vi "P5_PrintVIToHTML.vi"(11 "Inputs":string[](array[string])) -> (2 "Output/Failure":string, 3 "CLI Process Return Code":i32)   [LabVIEW 2026]
doc: "Slice 1.1 probe: Open VI Reference, Print VI To HTML to the path in arg, close the reference."
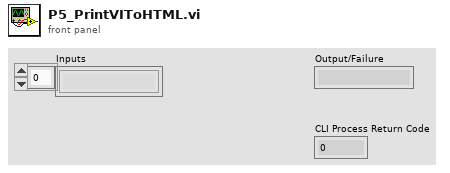
[diagram p1: front panel]
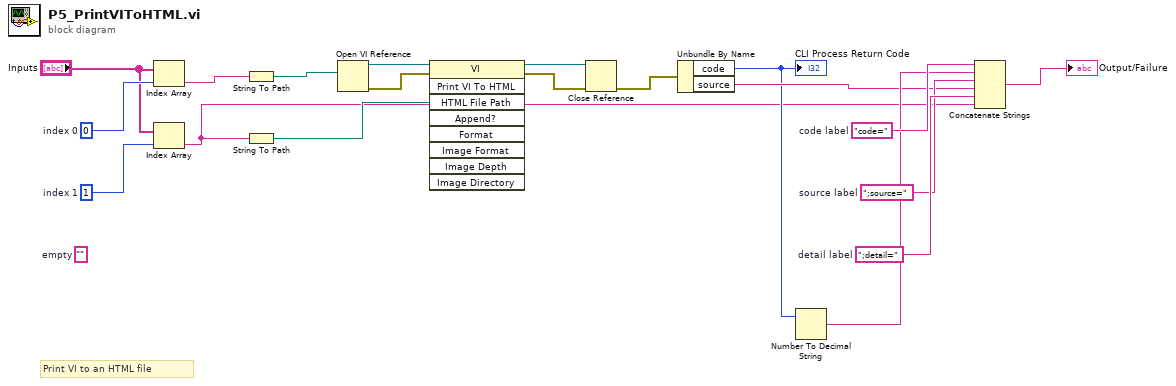
[diagram p0: block diagram]
diagram:
  w18 = ";detail="  # detail label
  w17 = ";source="  # source label
  w16 = "code="  # code label
  (unwired) ""  # empty
  w3 = 1  # index 1
  w2 = 0  # index 0
  # "Print VI to an HTML file"
  n1 = Index Array(array="Inputs", index=w2) -> (element=w4:string)
  n2 = Index Array(array="Inputs", index=w3) -> (element=w5:string)
  n3 = String To Path(string=w4) -> (path=w6:path)
  n4 = String To Path(string=w5) -> (path=w7:path)
  n5 = Open VI Reference(vi path=w6) -> (vi reference=w8:refnum<vi>, error out=w9:errorcluster)  [unwired: 5 in]
  n6 = invoke class="VI" method="Print VI To HTML"(reference=w8, error in=w9, "HTML File Path"=w7) -> (reference out=w10:refnum<vi>, error out=w11:errorcluster)  [unwired: 6 in, 7 out]
  n7 = Close Reference(reference=w10, error in (no error)=w11) -> (error out=w12:errorcluster)
  n8 = Unbundle By Name(w12) -> ("code"=w13:i32, "source"=w14:string)
  "CLI Process Return Code" <- w13
  n9 = Number To Decimal String(number=w13) -> (decimal integer string=w15:string)  [unwired: 1 in]
  n10 = Concatenate Strings(w16, w15, w17, w14, w18, w5) -> (→"Output/Failure":string)
